vi "Host_NetworkStreams.vi"() -> ()   [LabVIEW 2025]
uses:
  <vilib>/dex/Flush And Wait Empty Condition.ctl
  <vilib>/Analysis/NI_AALBase.lvlib
panel:
  out "error out":errorcluster
  out "Waveform Graph":dbl[][](graph)
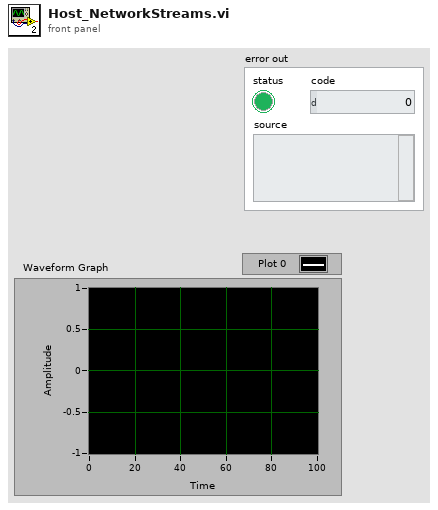
[diagram p1: front panel]
types:
  T1 = typedef "Flush And Wait Empty Condition.ctl" = u8
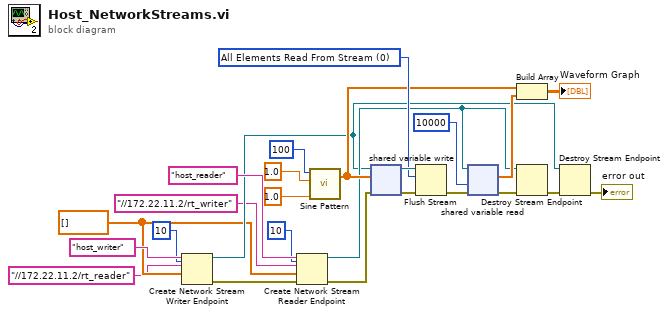
[diagram p0: block diagram]
diagram:
  w5 = dbl[] []
  w17 = T1 0 items=["All Elements Read From Stream", "All Elements Available for Reading"] ("wait condition")
  n1 = Create Network Stream Writer Endpoint(7:10 ("writer buffer size"), 9:w5, 10:"//172.22.11.2/rt_reader" ("reader url"), 11:"host_writer" ("writer name")) -> (0:w22:errorcluster, 3:w7:refnum<k21>)  [unwired: 3 in]
  n2 = Create Network Stream Reader Endpoint(7:10 ("reader buffer size"), 8:w22, 9:w5, 10:"//172.22.11.2/rt_writer" ("writer url"), 11:"host_reader" ("writer name")) -> (0:w19:errorcluster, 3:w8:refnum<k21>)  [unwired: 2 in]
  n3 = call <vilib>:"Sine Pattern.vi"("cycles"=1.0, "amplitude"=1.0, "samples"=100) -> ("Sinusoidal Pattern"=w12:dbl[])  [unwired: 1 in, 1 out]
  n4 = shared-variable-write(w7, w19, w12) -> (w18:refnum<k21>, w16:errorcluster)  [unwired: 1 in, 1 out]
  n5 = Flush Stream(8:w16, 10:w17, 11:w18) -> (0:w15:errorcluster)  [unwired: 1 in, 2 out]
  n6 = shared-variable-read(w8, w15, 10000 ("timeout ms (-1)")) -> (w10:errorcluster, w13:dbl[])  [unwired: 2 out]
  n7 = Build Array(w12, w13) -> (→"Waveform Graph":dbl[][])
  n8 = Destroy Stream Endpoint(8:w10, 11:w8) -> (0:w9:errorcluster)
  n9 = Destroy Stream Endpoint(8:w9, 11:w7) -> (0:→"error out":errorcluster)
